vi "Configure.vi"(8 "error in (no error)":errorcluster, 9 "bit timing":T1, 10 "config":T2={"connection"={"host"="", "channel"=2, "cert path"=path "/home/lvuser/cansub_root_cert.crt"}, "bit rates"={"nominal bit rate"=500000, "nominal sample point"=80.0, "data bit rate"=2000000, "data sample point"=80.0}, "listen only"=FALSE, "filters"=[], "read mode"=enum."Poll", "max bytes per read"=4096, "reader FIFO depth"=0, "reader priority"=0, "ownership"=enum."Direct"} {"filters"."f2" format="%.0x"; "filters"."f1" format="%.0x"}, 11 "channel in":refnum<class "CANsub_DirectChannel.lvclass">) -> (0 "error out":errorcluster, 3 "channel out":refnum<class "CANsub_DirectChannel.lvclass">)   [LabVIEW 2021, in "CANsub_API.lvlib" / "CANsub_DirectChannel.lvclass"]
doc: "Direct: stores config and bit timing; state = Closed. Called only by Init."
uses:
  CANsub_DirectChannel.lvclass
  CANsub_DirectChannel.lvclass/CANsub_DirectChannel.ctl
  Typedefs/CANsub_State.ctl
  CANsub_API.lvlib
  common/Typedefs/Bit_Timing.ctl
  common/CANsub_Common.lvlib
  Typedefs/CANsub_Status.ctl
  common/Typedefs/CANsub_connection.ctl
  common/Typedefs/CANsub_Bit_Rates.ctl
  Typedefs/CANsub_Filter.ctl
  Typedefs/CANsub_Read_Mode.ctl
  Typedefs/CANsub_Ownership.ctl
  Typedefs/CANsub_Config.ctl
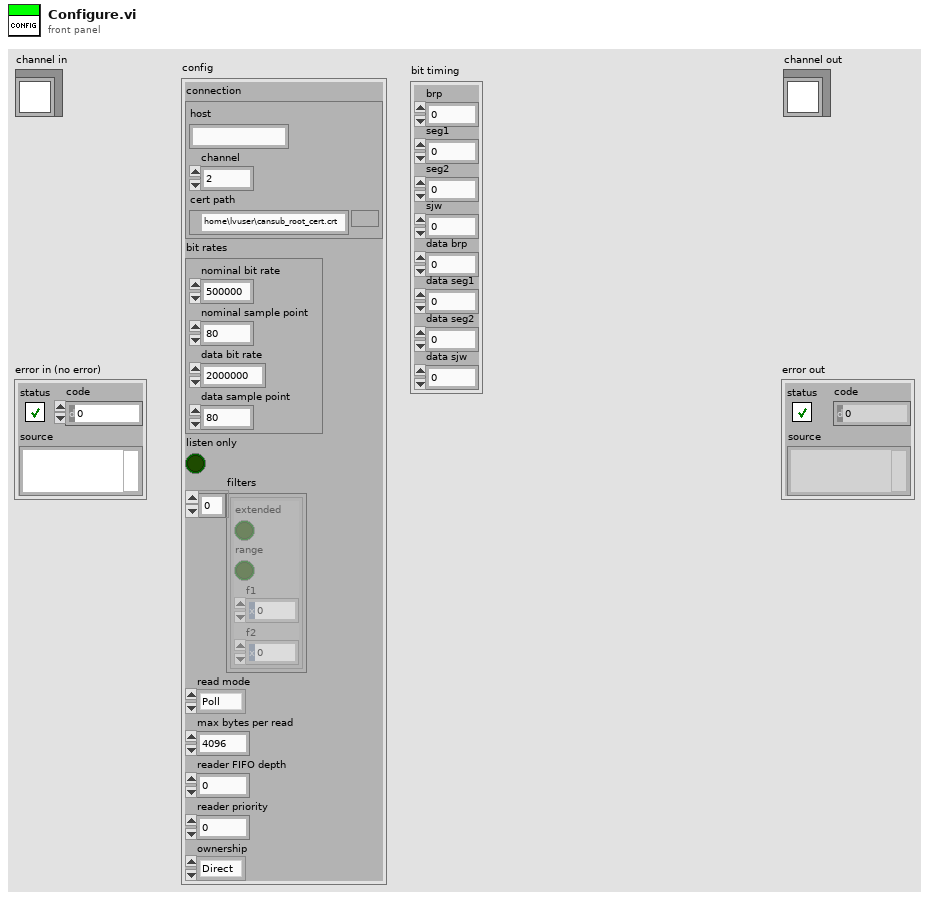
[diagram p1: front panel]
types:
  T1 = typedef "CANsub_Common.lvlib/Bit_Timing.ctl" = cluster{"brp":u16, "seg1":u16, "seg2":u16, "sjw":u16, "data brp":u16, "data seg1":u16, "data seg2":u16, "data sjw":u16}
  T2 = typedef "CANsub_API.lvlib/CANsub_Config.ctl" = cluster{"connection":T3, "bit rates":T4, "listen only":bool, "filters":T5[], "read mode":T6, "max bytes per read":i32, "reader FIFO depth":i32, "reader priority":i32, "ownership":T7}
  T3 = typedef "CANsub_Common.lvlib/CANsub_connection.ctl" = cluster{"host":string, "channel":u8, "cert path":path}
  T4 = typedef "CANsub_Common.lvlib/CANsub_Bit_Rates.ctl" = cluster{"nominal bit rate":u32, "nominal sample point":dbl, "data bit rate":u32, "data sample point":dbl}
  T5 = typedef "CANsub_API.lvlib/CANsub_Filter.ctl" = cluster{"extended":bool, "range":bool, "f1":u32, "f2":u32}
  T6 = typedef "CANsub_API.lvlib/CANsub_Read_Mode.ctl" = enum16{"Poll", "Reader"}
  T7 = typedef "CANsub_API.lvlib/CANsub_Ownership.ctl" = enum16{"Direct", "Shared"}
  T8 = typedef "CANsub_API.lvlib/CANsub_State.ctl" = enum16{"Closed", "Open", "Lost"}
  T9 = typedef "CANsub_API.lvlib/CANsub_Status.ctl" = cluster{"state":T8, "frames read":u32, "frames written":u32, "crc errors":u32, "decode errors":i32, "pings":u32, "FIFO overflows":u32, "reopens":u32, "nodelay":i32, "api version":string, "lib version":u32, "bit timing":T1, "last error":errorcluster}
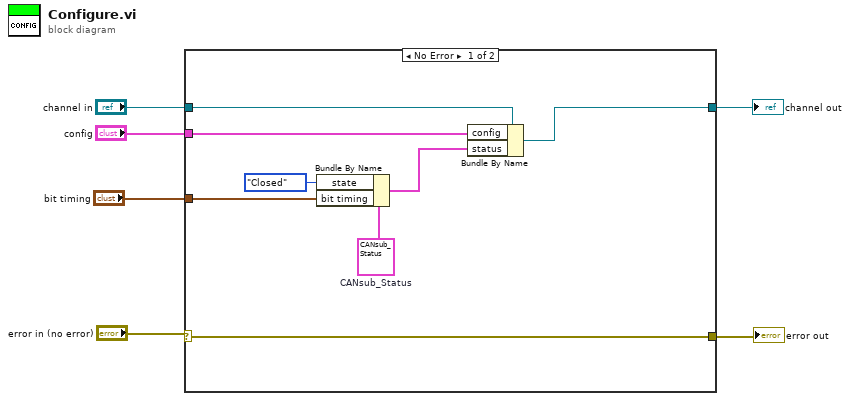
[diagram p0: block diagram]
diagram:
  n1 = case shown="No Error" "error in (no error)" {
    selector: "error in (no error)" -> [w7 w16]
    tunnel: [w7 w16] -> w5
    tunnel: [w11 w15] -> w4
    tunnel: "channel in" -> [w13 w15]
    tunnel: "config" -> [w12 _]
    tunnel: "bit timing" -> [w10 _]
    frame No Error {
      w14 = T9 {"state"=enum."Closed", "frames read"=0, "frames written"=0, "crc errors"=0, "decode errors"=0, "pings"=0, "FIFO overflows"=0, "reopens"=0, "nodelay"=0, "api version"="", "lib version"=0, "bit timing"={"brp"=0, "seg1"=0, "seg2"=0, "sjw"=0, "data brp"=0, "data seg1"=0, "data seg2"=0, "data sjw"=0}, "last error"={"status"=FALSE, "code"=0, "source"=""}}  # CANsub_Status
      n2 = Bundle By Name(cluster=w14, "state"=CANsub_State."Closed", "bit timing"=w10) -> (w8:T9)
      n3 = Bundle By Name(cluster=w13, "config"=w12, "status"=w8) -> (w11:refnum<class "CANsub_DirectChannel.lvclass">)
    }
    frame Error {
    }
  }
  "error out" <- w5
  "channel out" <- w4
